vi "Hex-String To String.vi"(11 "HEX-String":string) -> (3 "string":string)   [LabVIEW 2019, in "Language Selection.lvlib"]
doc: "- - -\nCopyright (c) 2026, Merecs Engineering GmbH"
uses:
  Language Selection.lvlib
panel:
  # "Connector Pane"
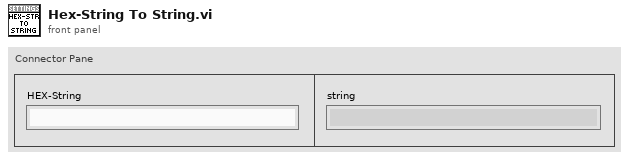
[diagram p1: front panel]
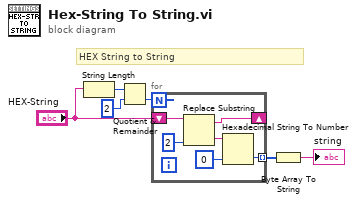
[diagram p0: block diagram]
diagram:
  # "HEX String to String"
  n1 = String Length(string="HEX-String") -> (length=w1:i32)
  n2 = Quotient & Remainder(x=w1, y=u64 2) -> (floor(x/y)=w4:u64)  [unwired: 1 out]
  n3 = for {
    N: w4 -> [_]
    shift-right: [w10] -> _
    shift-left: "HEX-String" -> [w12]
    tunnel: [w7] -> w3 mode=indexing
    n4 = Replace Substring(2:2 ("length (len. of substring)"), 5:w12) -> (0:w8:string, 1:w10:string)  [unwired: 2 in]
    n5 = Hexadecimal String To Number(string=w8, default (0uL)=u8 0 ("default (0 U32)")) -> (number=w7:u8)  [unwired: 1 in, 1 out]
  }
  n6 = Byte Array To String(unsigned byte array=w3) -> (string=→"string":string)
